vi "Power.vi"(8 "error in (no error)":errorcluster, 9 "Enable Drive":bool, 10 "Enable Axis":bool, 11 "SoftmotionAxis in":refnum<class "SoftmotionAxis.lvclass">) -> (0 "error out":errorcluster, 3 "SoftmotionAxis out":refnum<class "SoftmotionAxis.lvclass">)   [LabVIEW 2017, in "SoftmotionAxis.lvclass"]
uses:
  SoftmotionAxis.lvclass
  <resource>/objmgr/nimcai.rc
  <resource>/objmgr/nimotion.rc
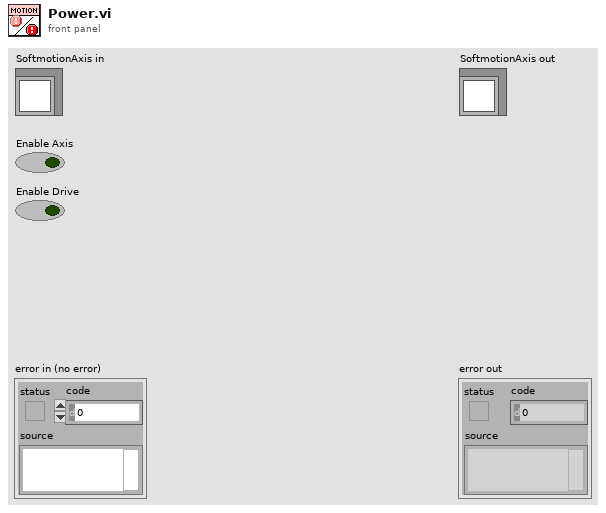
[diagram p1: front panel]
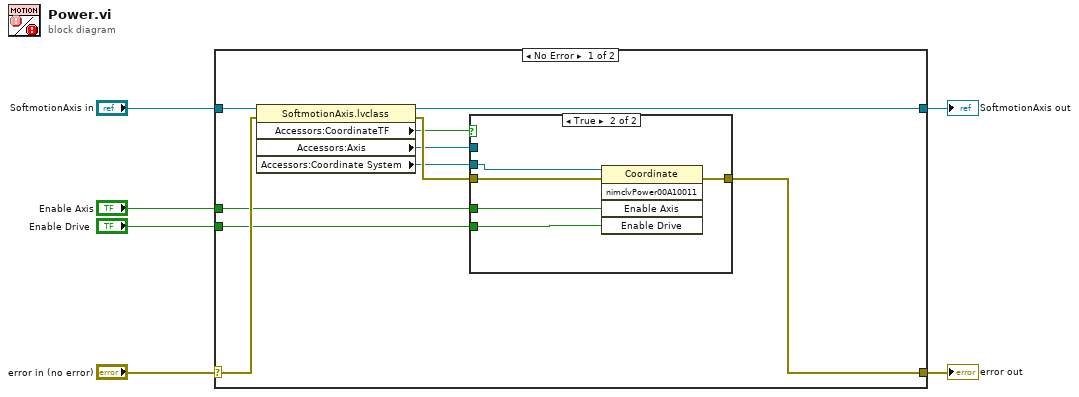
[diagram p0: block diagram]
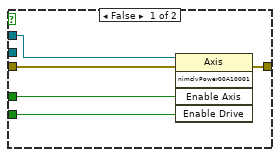
[diagram p2: hidden frame]
diagram:
  n1 = case shown="No Error" "error in (no error)" {
    selector: "error in (no error)" -> [w13 w28]
    tunnel: [w12 w28] -> w5
    tunnel: [w15 w27] -> w3
    tunnel: "SoftmotionAxis in" -> [w16 w27]
    tunnel: "Enable Axis" -> [w11 _]
    tunnel: "Enable Drive" -> [w10 _]
    frame No Error {
      n2 = property class="SoftmotionAxis.lvclass"(reference=w16, error in=w13) -> (reference out=w15:refnum<class "SoftmotionAxis.lvclass">, error out=w14:errorcluster, "Accessors:CoordinateTF"=w9:bool, "Accessors:Axis"=w8:refnum<k21>, "Accessors:Coordinate System"=w7:refnum<k21>)
      n3 = case shown="True" w9 {
        tunnel: w14 -> [w21 w26]
        tunnel: [w20 w25] -> w12
        tunnel: w11 -> [w19 w24]
        tunnel: w10 -> [w18 w23]
        tunnel: w8 -> [w17 _]
        tunnel: w7 -> [_ w22]
        frame False {
          n4 = invoke class="Axis" method="nimclvPower00A10001"(reference=w17, error in=w21, "Enable Axis"=w19, "Enable Drive"=w18) -> (error out=w20:errorcluster)  [unwired: 1 in, 4 out]
        }
        frame True {
          n5 = invoke class="Coordinate" method="nimclvPower00A10011"(reference=w22, error in=w26, "Enable Axis"=w24, "Enable Drive"=w23) -> (error out=w25:errorcluster)  [unwired: 1 in, 4 out]
        }
      }
    }
    frame Error {
    }
  }
  "error out" <- w5
  "SoftmotionAxis out" <- w3
